vi "10-2.vi"() -> ()   [LabVIEW 2025]
uses:
  <vilib>/Platform/TimedLoop/XDataNode/timing_clust.ctl
  <vilib>/Platform/TimedLoop/XDataNode/nitl_modes.ctl
  <vilib>/Platform/TimedLoop/XDataNode/wakeup.ctl
  <vilib>/eio/utilities/niEioResolveVilibRelativePath.vi
  <vilib>/rvi/interface/RandomDataEmulation/niFpgaRandomDataHandleErrors.vi
  <vilib>/rvi/Memory/Memory_Emulation/nirvimemoryFastEmulation.vi
  <vilib>/rvi/Memory/Memory_Emulation/nirvimemoryEmulation.vi
  <vilib>/rvi/Emulation/niFpgaEmulationIsFPGAContextNoSignature.vi
  <vilib>/rvi/DataTransferAndStorage/Container/Common/niFpgaContainerGetUniqueNameForEmu.vi
  <vilib>/rvi/Emulation/niFpgaProcessEmulError.vi
  <vilib>/rvi/Emulation/niFpgaSctlEmulationGetInTimedLoop.vi
  <vilib>/rvi/errors/nirviReportUnexpectedCaseInternalError (U32).vi
  <vilib>/rvi/Emulation/niFpgaEmulationReportErrorSimple.vi
  <vilib>/rvi/Emulation/niFpgaGetClockAttributes.vi
  <vilib>/rvi/Emulation/niFpgaCriticalErrorInLSC.vi
  <vilib>/rvi/linearAlgebra/MatrixMultiply/simVIs/SubVI/nifxpla_MatrixMultiply_SimMatrixSizes.vi
  <vilib>/rvi/linearAlgebra/MatrixMultiply/simVIs/SubVI/nifxpla_MatrixMultiply_Sim4WireAdapterVector.vi
  <vilib>/rvi/linearAlgebra/MatrixMultiply/simVIs/SubVI/nifxpla_MatrixMultiply_SimFrameHandShake.vi
  <vilib>/rvi/linearAlgebra/MatrixMultiply/simVIs/SubVI/nifxpla_MatrixMultiply_SimEndlessCounter.vi
  <vilib>/rvi/linearAlgebra/MatrixMultiply/simVIs/SubVI/nifxpla_MatrixMultiply_SimVectorDataBuffer.vi
  <vilib>/rvi/ClientSDK/Core/DevComputerLib/Private/Multiply(dfxp64).vi
  <vilib>/rvi/ClientSDK/Core/DevComputerLib/Private/Dfxp128ToDfxp256.vi
  <vilib>/rvi/ClientSDK/Core/DevComputerLib/Private/Add(dfxp256).vi
  <vilib>/rvi/ClientSDK/Core/DevComputerLib/Private/Subtract(dfxp256).vi
  <vilib>/rvi/ClientSDK/Core/DevComputerLib/Private/ToDfxp64(dfxp256).vi
  <vilib>/rvi/DataTransferAndStorage/Container/XNode/niFpgaContainer.xnode
  <vilib>/rvi/interface/RandomDataEmulation/nirviRandomDataFpgaReadWriteTemplate.vi
  <vilib>/platform/TimedLoop/XDataNode/XDataNode.xnode
  <vilib>/rvi/linearAlgebra/MatrixMultiply/XNode/nifxpla_MatrixMultiply.xnode
  <vilib>/rvi/linearAlgebra/MatrixMultiply/simVIs/nifxpla_MatrixMultiply_SimTemplateEinEout.vi
  <vilib>/rvi/linearAlgebra/MatrixMultiply/simVIs/nifxpla_MatrixMultiply_SimTemplateEinVout.vi
  <vilib>/rvi/linearAlgebra/MatrixMultiply/simVIs/nifxpla_MatrixMultiply_SimTemplateVinEout.vi
  <vilib>/rvi/linearAlgebra/MatrixMultiply/simVIs/nifxpla_MatrixMultiply_SimTemplateVinVout.vi
  <vilib>/Platform/TimedLoop/XDataNode/XDNodeRunTimeDep.lvlib
panel:
  out "Latency":u32
  out "Cycle Count":i32
  out "C1":fxp<+/-,32,16>[](array[numeric])
  out "C1+B":fxp<+/-,33,17>[](array[numeric])
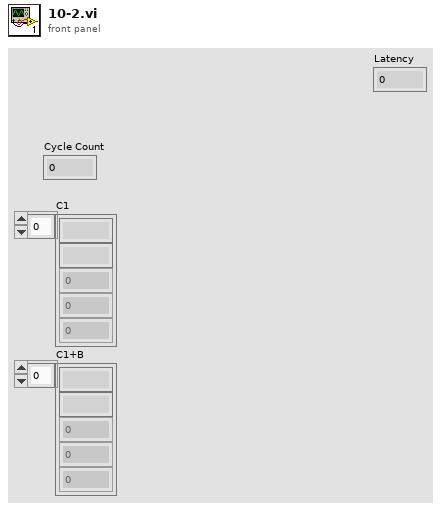
[diagram p1: front panel]
types:
  T1 = typedef "XDNodeRunTimeDep.lvlib/timing_clust.ctl" = cluster{"Expected End [f-1]":u64, "Actual End [f-1]":u64, "Finished Late? [f-1]":bool, "Expected End [i-1]":u64, "Actual End [i-1]":u64, "Finished Late? [i-1]":bool, "Expected Start [i]":u64, "Actual Start [i]":u64, "Expected Start [f]":u64, "Actual Start [f]":u64, "Source Name":string, "Structure Name":string, "Period":i64, "Deadline":i64, "Offset":i64, "Start":i64, "Priority":i32, "Timeout":i32, "Mode":T2, "Wakeup Reason":T3, "Error":errorcluster, "Source Type":string, "Secondary Source Type":string, "Global End Time":u64, "Global Start Time":u64, "Frame Duration":u64, "Iteration Duration":u64, "Assigned CPU":i32, "I/O Scan Engine Mode":u32}
  T2 = typedef "XDNodeRunTimeDep.lvlib/nitl_modes.ctl" = enum32{"No Change", "Process missed periods, maintain original phase", "Discard missed periods, maintain original phase", "Process missed periods, ignore original phase", "Discard missed periods, ignore original phase"}
  T3 = typedef "XDNodeRunTimeDep.lvlib/wakeup.ctl" = enum32{"Normal", "Aborted", "Asynchronous wakeup", "Timing source error", "Timed loop error", "Timeout"}
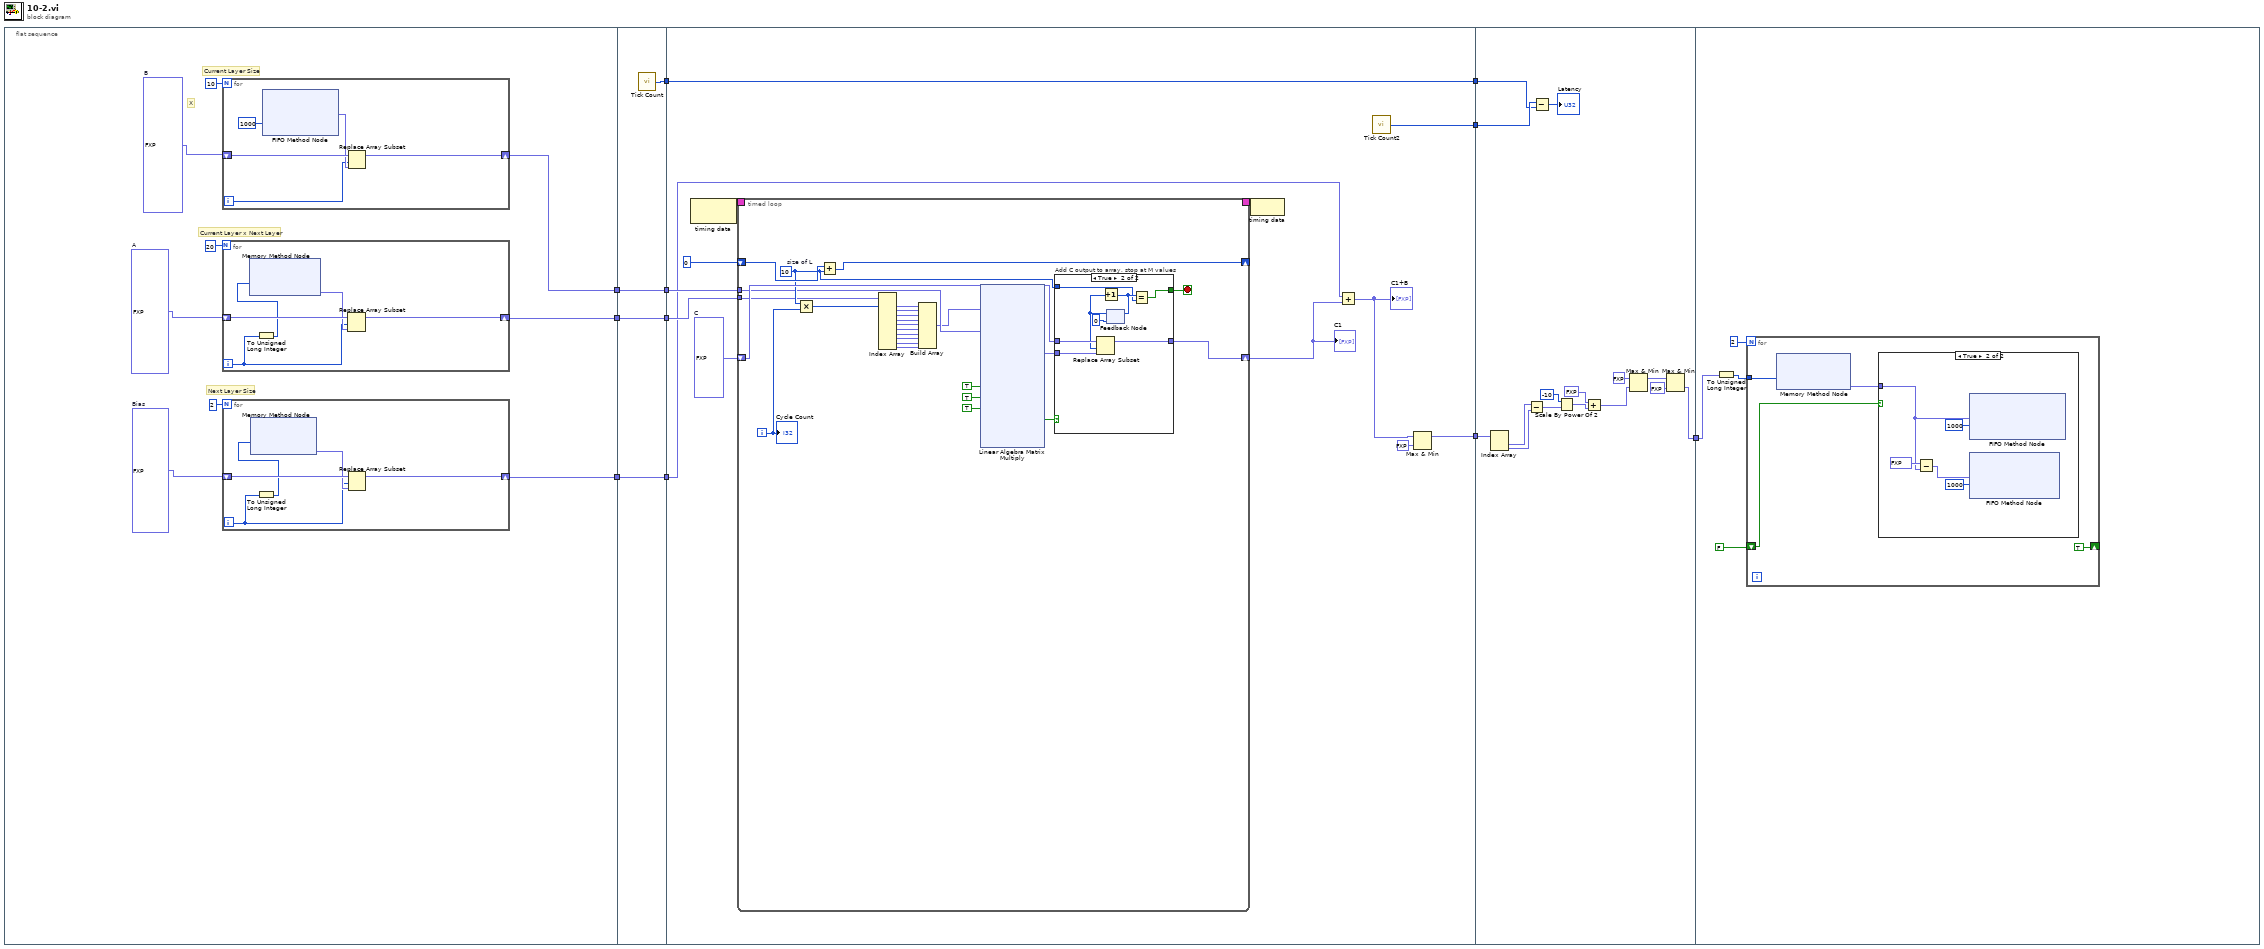
[diagram p0: block diagram]
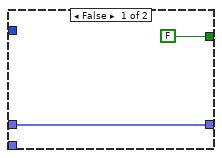
[diagram p2: hidden frame]
diagram:
  n1 = flat-sequence {
    tunnel: [w16] -> w7
    tunnel: [w13] -> w5
    tunnel: [w12] -> w2
    tunnel: [w39] -> w11
    tunnel: [w38] -> w8
    tunnel: w7 -> [w38]
    tunnel: [w37] -> w6
    tunnel: w5 -> [w37]
    tunnel: w2 -> [w36]
    tunnel: [w36] -> w1
    tunnel: [w52] -> w10
    tunnel: [w51] -> w9
    tunnel: [w49] -> w4
    tunnel: w11 -> [w52]
    tunnel: w8 -> [w43]
    tunnel: w6 -> [w40]
    tunnel: w1 -> [w41]
    tunnel: w10 -> [w106]
    tunnel: w9 -> [w107]
    tunnel: w4 -> [w104]
    tunnel: [w93] -> w3
    tunnel: w3 -> [w109]
    frame #0 {
      w14 = fxp<+/-,32,16>[] [0.0, 0.0]  # Bias
      w17 = fxp<+/-,32,16>[] [0.0, 0.0, 0.0, 0.0, 0.0, 0.0, 0.0, 0.0, 0.0, 0.0, 0.0, 0.0, 0.0, 0.0, 0.0, 0.0, 0.0, 0.0, 0.0, 0.0]  # A
      w19 = fxp<+/-,32,16>[] [0.0, 0.0, 0.0, 0.0, 0.0, 0.0, 0.0, 0.0, 0.0, 0.0]  # B
      # "Next Layer Size"
      # "Current Layer Size"
      # "Current Layer x Next Layer"
      # "X"
      n2 = for {
        N: 20 -> [_]
        shift-right: [w29] -> w12
        shift-left: w17 -> [w30]
        i -> [w27]
        n3 = To Unsigned Long Integer(number=w27) -> (unsigned 32bit integer=w26:u32)
        n4 = xnode ("Memory Method Node")("Address"=w26) -> ("Data"=w28:fxp<+/-,32,16>)  [unwired: 1 in, 1 out]
        n5 = Replace Array Subset(array=w30, new element=w28, index=w27) -> (w29:fxp<+/-,32,16>[])
      }
      n6 = for {
        N: 10 -> [_]
        shift-right: [w32] -> w16
        shift-left: w19 -> [w34]
        i -> [w31]
        n7 = xnode ("FIFO Method Node")("Timeout"=1000) -> ("Element"=w33:fxp<+/-,32,16>)  [unwired: 1 in, 2 out]
        n8 = Replace Array Subset(array=w34, new element=w33, index=w31) -> (w32:fxp<+/-,32,16>[])
      }
      n9 = for {
        N: 2 -> [_]
        shift-right: [w24] -> w13
        shift-left: w14 -> [w25]
        i -> [w22]
        n10 = To Unsigned Long Integer(number=w22) -> (unsigned 32bit integer=w21:u32)
        n11 = xnode ("Memory Method Node")("Address"=w21) -> ("Data"=w23:fxp<+/-,32,16>)  [unwired: 1 in, 1 out]
        n12 = Replace Array Subset(array=w25, new element=w23, index=w22) -> (w24:fxp<+/-,32,16>[])
      }
    }
    frame #1 {
      n13 = call "Tick Count"() -> ("Tick Count(Ticks)"=w39:u32)
    }
    frame #2 {
      w46 = fxp<+/-,32,16>[] [0.0, 0.0]  # C
      n14 = node-c288() -> (w48:T1)  [unwired: 1 in]
      n15 = timed-loop {
        timing: w48 -> [_]
        timing-out: [_] -> w47
        shift-right: [w77] -> w44
        shift-left: w46 -> [w76]
        shift-right: [w70] -> _
        shift-left: 0 ("length") -> [w71]
        tunnel: w41 -> [w55]
        tunnel: w43 -> [w54]
        i -> [w57]
        stop <- w75 stop-if-true
        w56 = 10  # size of L
        n16 = Multiply(x=w56, y=w57) -> (x*y=w68:i32)
        n17 = Add(x=w71, y=w56) -> (x+y=w70:i32)
        n18 = Index Array(array=w55, index #1=w68) -> (element #1=w67:fxp<+/-,32,16>, element #2=w66:fxp<+/-,32,16>, element #3=w65:fxp<+/-,32,16>, element #4=w64:fxp<+/-,32,16>, element #5=w63:fxp<+/-,32,16>, element #6=w62:fxp<+/-,32,16>, element #7=w61:fxp<+/-,32,16>, element #8=w60:fxp<+/-,32,16>, element #9=w59:fxp<+/-,32,16>, element #10=w58:fxp<+/-,32,16>)  [unwired: 9 in]
        n19 = Build Array(w67, w66, w65, w64, w63, w62, w61, w60, w59, w58) -> (w53:fxp<+/-,32,16>[])
        n20 = xnode ("Linear Algebra Matrix Multiply")("ar"=w53, "br"=w54, "a valid"=TRUE, "b valid"=TRUE, "ready for output (T)"=TRUE) -> ("cr"=w73:fxp<+/-,64,36>[], "output valid"=w69:bool)  [unwired: 2 in, 4 out]
        n21 = case "Add C output to array, stop at M values" shown="True" w69 {
          tunnel: w73 -> [_ w84]
          tunnel: [w80 w87] -> w77
          tunnel: w76 -> [w80 w88]
          tunnel: [FALSE w85] -> w75
          tunnel: w56 -> [_ w81]
          frame False {
          }
          frame True {
            n22 = feedback #1(0 ("x")) -> (w83:i32)
            n23 = Replace Array Subset(array=w88, new element=w84, index=w83) -> (w87:fxp<+/-,32,16>[])
            n24 = Increment(x=w83) -> (x+1=w82:i32)
            n25 = feedback-in #1(w82) -> ()
            n26 = Equal?(x=w82, y=w81) -> (x = y?=w85:bool)
          }
        }
        "Cycle Count" <- w57
      }
      "C1" <- w44
      n27 = node-c288(w47) -> ()
      n28 = Add(x=w40, y=w44) -> (x+y=w42:fxp<+/-,33,17>[])
      "C1+B" <- w42
      n29 = call "Tick Count2"() -> ("Tick Count(Ticks)"=w51:u32)
      n30 = Max & Min(x=w42, y=fxp<+,1,1> 0.0) -> (max(x,y)=w49:fxp<+/-,33,17>[])  [unwired: 1 out]
    }
    frame #3 {
      n31 = Index Array(array=w104) -> (element #1=w95:fxp<+/-,33,17>, element #2=w94:fxp<+/-,33,17>)  [unwired: 2 in]
      n32 = Subtract(x=w95, y=w94) -> (x-y=w100:fxp<+/-,34,18>)
      n33 = Subtract(x=w107, y=w106) -> (x-y=→"Latency":u32)
      n34 = Scale By Power Of 2(n=i16 -10, x=w100) -> (x*2^n=w101:fxp<+/-,34,18>)
      n35 = Add(x=fxp<+,1,9> 256.0, y=w101) -> (x+y=w102:fxp<+/-,35,19>)
      n36 = Max & Min(x=fxp<+,1,1> 0.0, y=w102) -> (max(x,y)=w103:fxp<+/-,35,19>)  [unwired: 1 out]
      n37 = Max & Min(x=w103, y=fxp<+,9,9> 511.0) -> (min(x,y)=w93:fxp<+/-,35,19>)  [unwired: 1 out]
    }
    frame #4 {
      n38 = To Unsigned Long Integer(number=w109) -> (unsigned 32bit integer=w108:u32)
      n39 = for {
        N: 2 -> [_]
        tunnel: w108 -> [w115]
        shift-right: [TRUE] -> _
        shift-left: FALSE -> [w114]
        n40 = xnode ("Memory Method Node")("Address"=w115) -> ("Data"=w112:fxp<+/-,32,16>)  [unwired: 1 in, 1 out]
        n41 = case shown="True" w114 {
          tunnel: w112 -> [_ w116]
          frame False {
          }
          frame True {
            n42 = Subtract(x=fxp<+,1,16> 32768.0, y=w116) -> (x-y=w120:fxp<+,33,17>)
            n43 = xnode ("FIFO Method Node")("Element"=w116, "Timeout"=1000) -> ()  [unwired: 1 in, 2 out]
            n44 = xnode ("FIFO Method Node")("Element"=w120, "Timeout"=1000) -> ()  [unwired: 1 in, 2 out]
          }
        }
      }
    }
  }
